vi "Read Default Tasks.vi"(8 "error in":errorcluster, 11 "Project Store in":refnum<class "Project Store.lvclass">) -> (0 "error out":errorcluster, 2 "Task Names":string[](array[string]), 3 "Project Store out":refnum<class "Project Store.lvclass">)   [LabVIEW 2026]
doc: "Returns the default task names - the [Default Tasks] section of Settings.ini in the data folder of the Project Store - in the order of the file, which is Task_N order: Migrate v1 Data.vi writes that section from the version-1 [Default] project as Task_0..n.\n\nThe data folder is read from the store as a Project Store-INI (To More Specific Class). When the store is not a Project Store-INI, or Settings.ini or its [Default Tasks] section is missing, Task Names is empty and no error is returned.\n\nInputs: Project Store in; error in.\nOutputs: Task Names; Project Store out (the store passed through); error out.\n\nGenerated by: Claude"
uses:
  Storage/Project Store/Project Store.lvclass
  Storage/Project Store-INI/Project Store-INI.lvclass
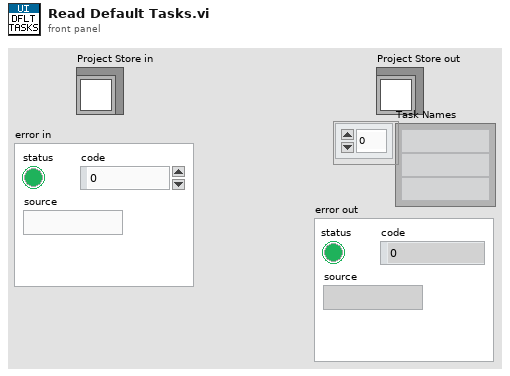
[diagram p1: front panel]
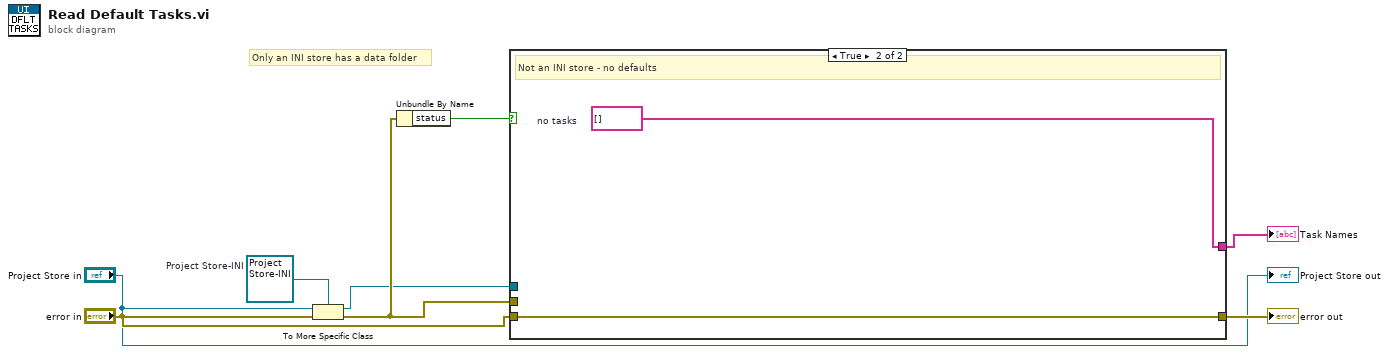
[diagram p0: block diagram]
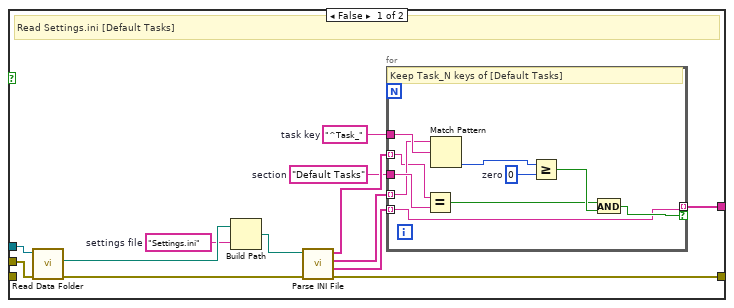
[diagram p2: hidden frame]
diagram:
  w5 = refnum<class "Project Store-INI.lvclass"> refnum  # Project Store-INI
  # "Only an INI store has a data folder"
  n1 = To More Specific Class(target class=w5, reference="Project Store in", error in="error in") -> (specific class reference=w6:refnum<class "Project Store-INI.lvclass">, error out=w7:errorcluster)
  n2 = Unbundle By Name(w7) -> ("status"=w8:bool)
  n3 = case shown="True" w8 {
    tunnel: "error in" -> [_ w32]
    tunnel: [w21 w33] -> w3
    tunnel: w6 -> [w9 _]
    tunnel: w7 -> [w10 _]
    tunnel: [w20 w32] -> w4
    frame False {
      w13 = "^Task_"  # task key
      w12 = "Default Tasks"  # section
      w11 = "Settings.ini"  # settings file
      # "Read Settings.ini [Default Tasks]"
      n4 = call-dynamic "Read Data Folder.vi"("error in (no error)"=w10, "Project Store-INI in"=w9) -> ("error out"=w15:errorcluster, "Data Folder"=w14:path)  [unwired: 7 in, 1 out]
      n5 = Build Path(base path=w14, name or relative path=w11) -> (appended path=w16:path)
      n6 = call "Parse INI File.vi"("error in (no error)"=w15, "File Path"=w16) -> ("error out"=w20:errorcluster, "Values"=w19:string[], "Keys"=w18:string[], "Sections"=w17:string[])  [unwired: 6 in]
      n7 = for {
        tunnel: w12 -> [w25]
        tunnel: w13 -> [w26]
        tunnel: w17 -> [w22] mode=indexing
        tunnel: w18 -> [w23] mode=indexing
        tunnel: w19 -> [w24] mode=indexing
        tunnel: [w24] -> w21 mode=indexing if=w31
        w27 = 0  # zero
        # "Keep Task_N keys of [Default Tasks]"
        n8 = Equal?(x=w22, y=w25) -> (x = y?=w28:bool)
        n9 = Match Pattern(string=w23, regular expression=w26) -> (offset past match=w29:i32)  [unwired: 1 in, 3 out]
        n10 = Greater Or Equal?(x=w29, y=w27) -> (x >= y?=w30:bool)
        n11 = And(x=w28, y=w30) -> (x .and. y?=w31:bool)
      }
    }
    frame True {
      w33 = string[] []  # no tasks
      # "Not an INI store - no defaults"
    }
  }
  "Task Names" <- w3
  "error out" <- w4
  "Project Store out" <- "Project Store in"
